vi "Send_UIWriteCtrlArray.vi"(7 "Value Signaling (F)":bool[](array[boolean]), 8 "error in":errorcluster, 9 "Control Data":variant[](array[variant]), 10 "Control Label":string[](array[string]), 11 "Queue in":refnum<queue>) -> (0 "error out":errorcluster)   [LabVIEW 2025, in "UI_Library.lvlib"]
uses:
  UI_Library.lvlib
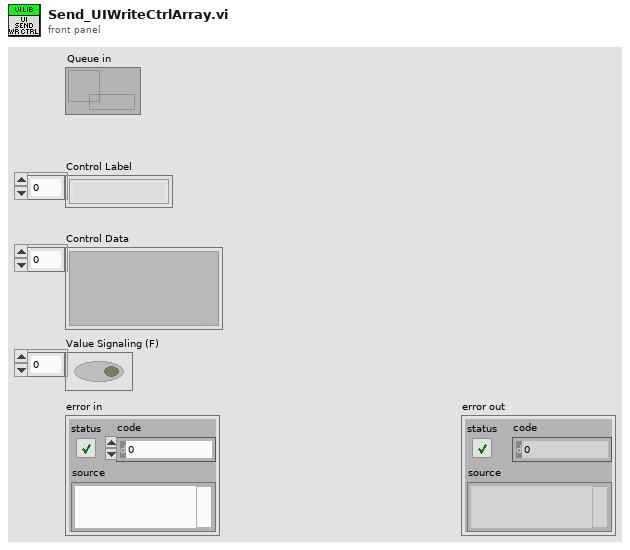
[diagram p1: front panel]
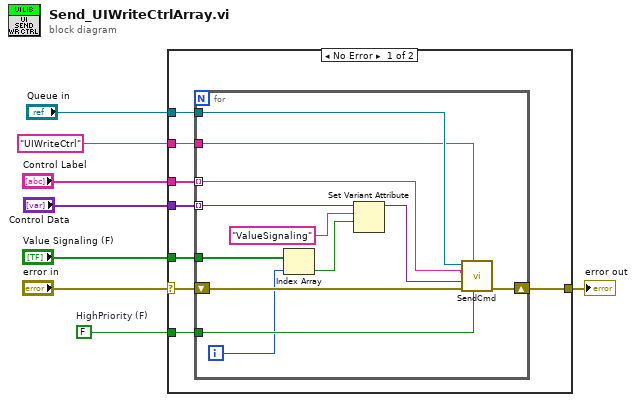
[diagram p0: block diagram]
diagram:
  w6 = FALSE  # HighPriority (F)
  n1 = case shown="No Error" "error in" {
    selector: "error in" -> [w15 w29]
    tunnel: "Queue in" -> [w16 _]
    tunnel: "Control Label" -> [w9 _]
    tunnel: "Control Data" -> [w11 _]
    tunnel: "UIWriteCtrl" ("UICmd") -> [w13 _]
    tunnel: w6 -> [w12 _]
    tunnel: [w14 w29] -> w8
    tunnel: "Value Signaling (F)" -> [w10 _]
    frame No Error {
      n2 = for {
        tunnel: w16 -> [w28]
        tunnel: w13 -> [w25]
        tunnel: w12 -> [w24]
        tunnel: w11 -> [w22] mode=indexing
        tunnel: w10 -> [w17]
        tunnel: w9 -> [w20] mode=indexing
        shift-right: [w26] -> w14
        shift-left: w15 -> [w27]
        i -> [w19]
        n3 = Index Array(array=w17, index=w19) -> (element=w18:bool)
        n4 = Set Variant Attribute(Variant=w22, name="ValueSignaling", value=w18) -> (Variant out=w21:variant)  [unwired: 1 in, 2 out]
        n5 = call "SendCmd.vi"("HighPriority (F)"=w24, "UICmd"=w25, "error in"=w27, "Control Data"=w21, "Control Label"=w20, "Queue in"=w28) -> ("error out"=w26:errorcluster)  [unwired: 5 in]
      }
    }
    frame Error {
    }
  }
  "error out" <- w8
